vi "move to Target Position.vi"(8 "error in (no error)":errorcluster, 11 "3D Controller in":refnum<class "3D Controller.lvclass">) -> (0 "error out":errorcluster, 3 "3D Controller out":refnum<class "3D Controller.lvclass">)   [LabVIEW 2023, in "FCC 3D Controller for BS.lvlib" / "3D Controller.lvclass"]
uses:
  3D Controller.lvclass
  3D Controller.lvclass/3D Controller.ctl
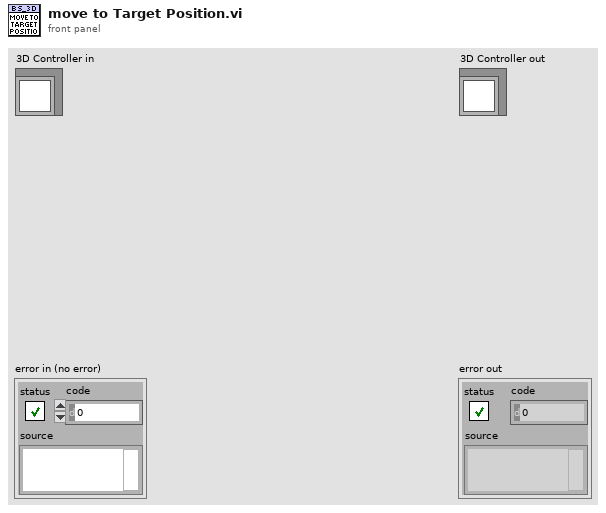
[diagram p1: front panel]
types:
  T1 = typedef "FCC 3D Controller for BS.lvlib/TYPE Protocol Char of Command.ctl" = cluster{"Header":string, "Axis No.":i32, "End":string}
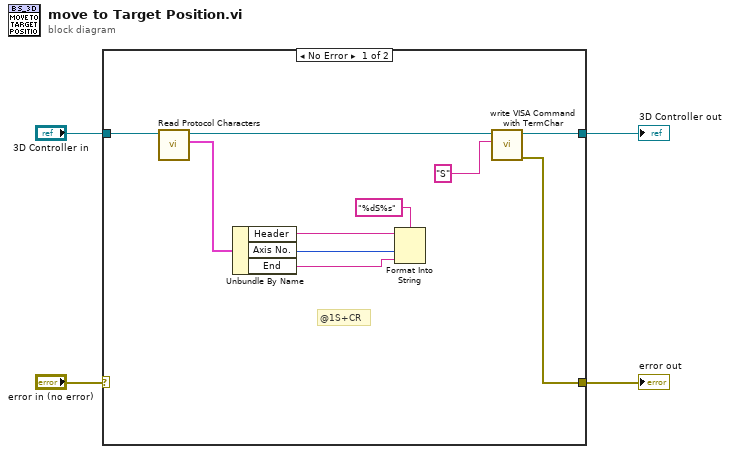
[diagram p0: block diagram]
diagram:
  n1 = case shown="No Error" "error in (no error)" {
    selector: "error in (no error)" -> [_ w16]
    tunnel: "3D Controller in" -> [w7 w15]
    tunnel: [w8 w16] -> w1
    tunnel: [w9 w15] -> w3
    frame No Error {
      # "@1S+CR"
      n2 = call "Read Protocol Characters.vi"("3D Controller in"=w7) -> ("Protocol Characters"=w13:T1, "3D Controller out"=w10:refnum<class "3D Controller.lvclass">)  [unwired: 8 in, 1 out]
      n3 = Unbundle By Name(w13) -> ("Header"=w12:string, "Axis No."=w11:i32, "End"=w6:string)
      n4 = Format Into String(format string="%dS%s", initial string=w12, w11, w6) -> ()  [unwired: 1 in, 2 out]
      n5 = call "write VISA Command with TermChar.vi"("Command String"="S", "3D Controller in"=w10) -> ("error out"=w8:errorcluster, "3D Controller out"=w9:refnum<class "3D Controller.lvclass">)  [unwired: 8 in]
    }
    frame Error {
    }
  }
  "error out" <- w1
  "3D Controller out" <- w3
